vi "PicoScope2000aSettings.vi"(0 "error in":errorcluster, 1 "Channel A Settings":T2 {"Analogue Offset" format="%#_6p"; "Range" items=["20 mV", "50 mV", "100 mV", "200 mV", "500 mV", "1 V", "2 V", "5 V", "10 V", "20 V"]; "Coupling" items=["AC", "DC"]}, 3 "Channel B Settings":T2 {"Range" items=["20 mV", "50 mV", "100 mV", "200 mV", "500 mV", "1 V", "2 V", "5 V", "10 V", "20 V"]; "Coupling" items=["AC", "DC"]}, 5 "handle in":i16, 7 "Channel C Settings":T2 {"Analogue Offset" format="%#_6p"; "Range" items=["20 mV", "50 mV", "100 mV", "200 mV", "500 mV", "1 V", "2 V", "5 V", "10 V", "20 V"]; "Coupling" items=["AC", "DC"]}, 9 "Channel D Settings":T2 {"Analogue Offset" format="%#_6p"; "Range" items=["20 mV", "50 mV", "100 mV", "200 mV", "500 mV", "1 V", "2 V", "5 V", "10 V", "20 V"]; "Coupling" items=["AC", "DC"]}, 11 "Trigger Settings":T4 {"Trigger Direction" items=["Rising", "Falling"]}, 12 "Port 0 Settings":T3 {"Logic Level" items=["1.5V TTL", "2.5V CMOS"]}, 13 "Device Info":T1, 14 "Port 1 Settings":T3 {"Logic Level" items=["1.5V TTL", "2.5V CMOS"]}, 15 "Max_adc":i16) -> (4 "error out":errorcluster, 6 "handle out":i16, 8 "Enabled Array":i16[](array[numeric]))   [LabVIEW 2009]
doc: "This VI is used to set up the oscilloscope. The inputs are clusters for setting channel and simple trigger settings. Advanced triggers can be set up using PicoScope3000aAdvancedTriggerSettings.vi"
uses:
  ps2000a.dll
  PicoScope2000aAnalogChannelSettings.ctl
  PicoScope2000aDigitalChannelSettings.ctl
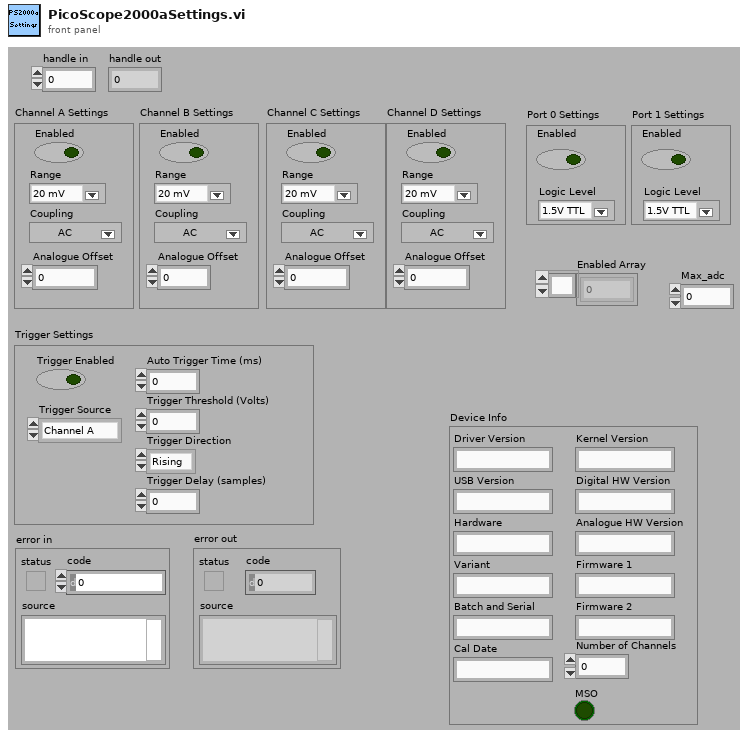
[diagram p1: front panel]
types:
  T1 = cluster{"Driver Version":string, "USB Version":string, "Hardware":string, "Variant":string, "Batch and Serial":string, "Cal Date":string, "Kernel Version":string, "Digital HW Version":string, "Analogue HW Version":string, "Firmware 1":string, "Firmware 2":string, "MSO":bool, "Number of Channels":i16}
  T2 = typedef "PicoScope2000aAnalogChannelSettings.ctl" = cluster{"Enabled":bool, "Coupling":i16, "Range":u16, "Analogue Offset":sgl}
  T3 = typedef "PicoScope2000aDigitalChannelSettings.ctl" = cluster{"Enabled":bool, "Logic Level":i16}
  T4 = cluster{"Trigger Enabled":bool, "Trigger Source":enum16{"Channel A", "Channel B", "Channel C", "Channel D", "Ext."}, "Trigger Threshold (Volts)":dbl, "Trigger Direction":u16, "Trigger Delay (samples)":u32, "Auto Trigger Time (ms)":i16}
  T5 = enum16{"Channel A", "Channel B", "Channel C", "Channel D", "Ext."}
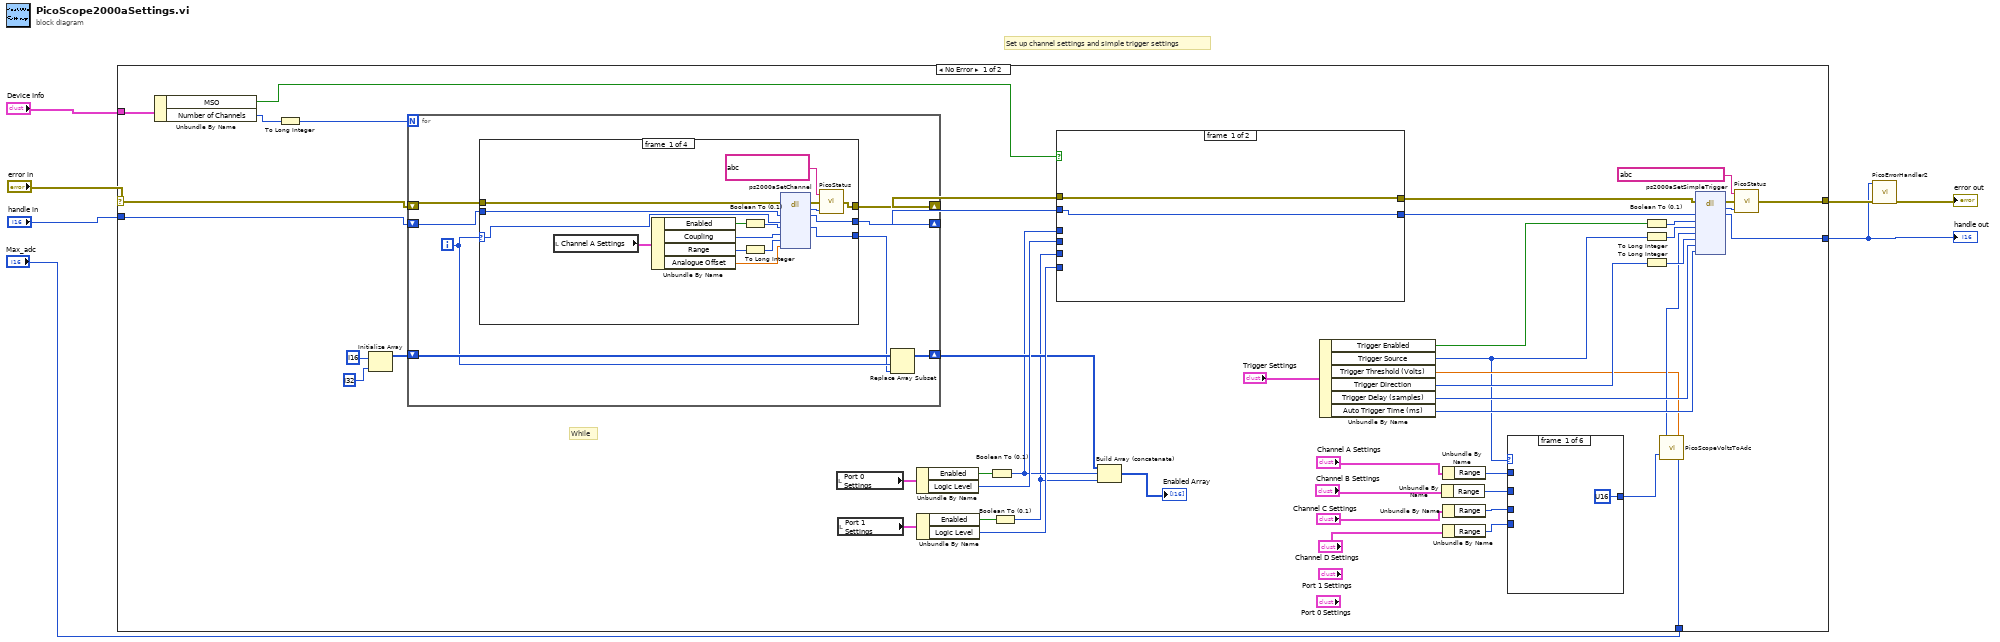
[diagram p0: block diagram]
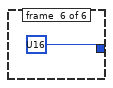
[diagram p6: hidden frame]
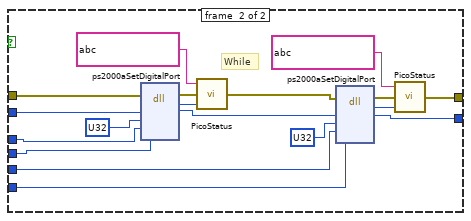
[diagram p7: hidden frame]
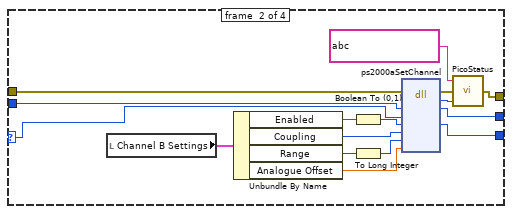
[diagram p8: hidden frame]
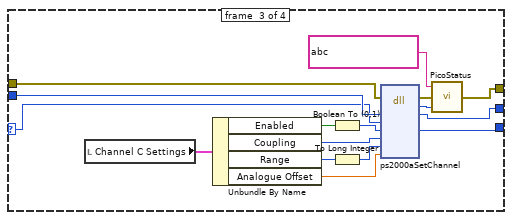
[diagram p9: hidden frame]
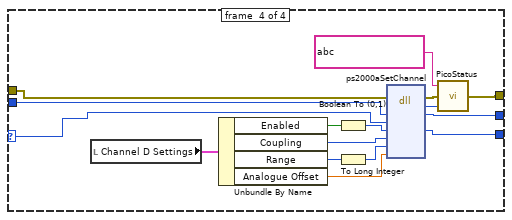
[diagram p10: hidden frame]
diagram:
  # "Set up channel settings and simple trigger settings"
  n1 = case shown="No Error" "error in" {
    selector: "error in" -> [w33 w155]
    tunnel: "handle in" -> [w32 w156]
    tunnel: [w9 w156] -> w2
    tunnel: "Max_adc" -> [w23 _]
    tunnel: "Device Info" -> [w25 _]
    tunnel: [w8 w155] -> w3
    frame #0 {
      # "While"
      n2 = Unbundle By Name(w25) -> ("MSO"=w24:bool, "Number of Channels"=w22:i16)
      n3 = To Long Integer(number=w22) -> (32bit integer=w11:i32)
      n4 = Initialize Array(i16 ? ("element"), i32 ? ("dimension size")) -> (w29:i16[])
      n5 = for {
        N: w11 -> [_]
        shift-right: [w90] -> w35
        shift-left: w33 -> [w89]
        shift-right: [w88] -> w34
        shift-left: w32 -> [w87]
        shift-right: [w83] -> w28
        shift-left: w29 -> [w86]
        i -> [w85]
        n6 = case shown="1" w85 {
          selector: w85 -> [w92 w108 w124 w140]
          tunnel: [w103 w119 w128 w144] -> w90
          tunnel: w89 -> [w102 w118 w126 w142]
          tunnel: w87 -> [w101 w117 w125 w141]
          tunnel: [w100 w116 w127 w143] -> w88
          tunnel: [w91 w107 w123 w139] -> w84
          frame #0 {
            n7 = local read "Channel A Settings"() -> (w93:T2)
            n8 = Unbundle By Name(w93) -> ("Enabled"=w96:bool, "Coupling"=w99:i16, "Range"=w94:u16, "Analogue Offset"=w98:sgl)
            n9 = Boolean To (0,1)(Boolean=w96) -> (0, 1=w97:i16)
            n10 = To Long Integer(number=w94) -> (32bit integer=w95:i32)
            n11 = dll-call lib="ps2000a.dll" fn="ps2000aSetChannel" ("ps2000a.dll:_ps3000_open_unit@0")(error in=w102, "handle"=w101, "channel"=w92, "enabled"=w97, "dc"=w99, "range"=w95, "analogueOffset"=w98) -> (error out=w105:errorcluster, "PICO_STATUS"=w104:u32, "handle"=w100:i16, "enabled"=w91:i16)  [unwired: 6 in, 1 out]
            n12 = call "PicoStatus.vi"("PICO STATUS"=w104, "error in"=w105, "source"=string ?) -> ("error out"=w103:errorcluster)
          }
          frame #1 {
            n13 = local read "Channel B Settings"() -> (w109:T2)
            n14 = Unbundle By Name(w109) -> ("Enabled"=w112:bool, "Coupling"=w115:i16, "Range"=w110:u16, "Analogue Offset"=w114:sgl)
            n15 = Boolean To (0,1)(Boolean=w112) -> (0, 1=w113:i16)
            n16 = To Long Integer(number=w110) -> (32bit integer=w111:i32)
            n17 = dll-call lib="ps2000a.dll" fn="ps2000aSetChannel" ("ps2000a.dll:_ps3000_open_unit@0")(error in=w118, "handle"=w117, "channel"=w108, "enabled"=w113, "dc"=w115, "range"=w111, "analogueOffset"=w114) -> (error out=w121:errorcluster, "PICO_STATUS"=w120:u32, "handle"=w116:i16, "enabled"=w107:i16)  [unwired: 6 in, 1 out]
            n18 = call "PicoStatus.vi"("PICO STATUS"=w120, "error in"=w121, "source"=string ?) -> ("error out"=w119:errorcluster)
          }
          frame #2 {
            n19 = local read "Channel C Settings"() -> (w138:T2)
            n20 = Unbundle By Name(w138) -> ("Enabled"=w135:bool, "Coupling"=w132:i16, "Range"=w137:u16, "Analogue Offset"=w133:sgl)
            n21 = Boolean To (0,1)(Boolean=w135) -> (0, 1=w134:i16)
            n22 = To Long Integer(number=w137) -> (32bit integer=w136:i32)
            n23 = dll-call lib="ps2000a.dll" fn="ps2000aSetChannel" ("ps2000a.dll:_ps3000_open_unit@0")(error in=w126, "handle"=w125, "channel"=w124, "enabled"=w134, "dc"=w132, "range"=w136, "analogueOffset"=w133) -> (error out=w130:errorcluster, "PICO_STATUS"=w131:u32, "handle"=w127:i16, "enabled"=w123:i16)  [unwired: 6 in, 1 out]
            n24 = call "PicoStatus.vi"("PICO STATUS"=w131, "error in"=w130, "source"=string ?) -> ("error out"=w128:errorcluster)
          }
          frame #3 {
            n25 = local read "Channel D Settings"() -> (w154:T2)
            n26 = Unbundle By Name(w154) -> ("Enabled"=w151:bool, "Coupling"=w148:i16, "Range"=w153:u16, "Analogue Offset"=w149:sgl)
            n27 = Boolean To (0,1)(Boolean=w151) -> (0, 1=w150:i16)
            n28 = To Long Integer(number=w153) -> (32bit integer=w152:i32)
            n29 = dll-call lib="ps2000a.dll" fn="ps2000aSetChannel" ("ps2000a.dll:_ps3000_open_unit@0")(error in=w142, "handle"=w141, "channel"=w140, "enabled"=w150, "dc"=w148, "range"=w152, "analogueOffset"=w149) -> (error out=w146:errorcluster, "PICO_STATUS"=w147:u32, "handle"=w143:i16, "enabled"=w139:i16)  [unwired: 6 in, 1 out]
            n30 = call "PicoStatus.vi"("PICO STATUS"=w147, "error in"=w146, "source"=string ?) -> ("error out"=w144:errorcluster)
          }
        }
        n31 = Replace Array Subset(array=w86, new element=w84, index=w85) -> (w83:i16[])
      }
      n32 = local read "Port 0 Settings"() -> (w42:T3)
      n33 = local read "Port 1 Settings"() -> (w40:T3)
      n34 = Unbundle By Name(w42) -> ("Enabled"=w43:bool, "Logic Level"=w39:i16)
      n35 = Unbundle By Name(w40) -> ("Enabled"=w41:bool, "Logic Level"=w38:i16)
      n36 = Boolean To (0,1)(Boolean=w43) -> (0, 1=w27:i16)
      n37 = Boolean To (0,1)(Boolean=w41) -> (0, 1=w26:i16)
      n38 = case shown="True" w24 {
        tunnel: w27 -> [_ w74]
        tunnel: w39 -> [_ w73]
        tunnel: w26 -> [_ w72]
        tunnel: w38 -> [_ w71]
        tunnel: [w64 w68] -> w37
        tunnel: [w63 w67] -> w36
        tunnel: w35 -> [w64 w66]
        tunnel: w34 -> [w63 w65]
        frame #0 {
        }
        frame #1 {
          # "While"
          n39 = dll-call lib="PS2000a.dll" fn="ps2000aSetDigitalPort"(error in=w66, "handle"=w65, "port"=u32 ? ("channel"), "enabled"=w74, "logicLevel"=w73) -> (error out=w82:errorcluster, "PICO_STATUS"=w80:u32, "handle"=w70:i16)  [unwired: 5 in, 1 out]
          n40 = call "PicoStatus.vi"("PICO STATUS"=w80, "error in"=w82, "source"=string ?) -> ("error out"=w69:errorcluster)
          n41 = dll-call lib="PS2000a.dll" fn="ps2000aSetDigitalPort"(error in=w69, "handle"=w70, "port"=u32 ? ("channel"), "enabled"=w72, "logicLevel"=w71) -> (error out=w78:errorcluster, "PICO_STATUS"=w76:u32, "handle"=w67:i16)  [unwired: 5 in, 1 out]
          n42 = call "PicoStatus.vi"("PICO STATUS"=w76, "error in"=w78, "source"=string ?) -> ("error out"=w68:errorcluster)
        }
      }
      n43 = Build Array (concatenate)(w28, w27, w26) -> (→"Enabled Array":i16[])
      n44 = Unbundle By Name("Trigger Settings") -> ("Trigger Enabled"=w50:bool, "Trigger Source"=w20:T5, "Trigger Threshold (Volts)"=w44:dbl, "Trigger Direction"=w53:u16, "Trigger Delay (samples)"=w52:u32, "Auto Trigger Time (ms)"=w51:i16)
      n45 = Unbundle By Name("Channel B Settings") -> ("Range"=w18:u16)
      n46 = Unbundle By Name("Channel A Settings") -> ("Range"=w19:u16)
      n47 = Unbundle By Name("Channel C Settings") -> ("Range"=w17:u16)
      n48 = Unbundle By Name("Channel D Settings") -> ("Range"=w16:u16)
      n49 = case shown="\"Channel A\"" w20 {
        tunnel: [u16 ? ("Range") w58 w59 w60 w61 u16 ? ("Range")] -> w21
        tunnel: w19 -> [_ w58 _ _ _ _]
        tunnel: w18 -> [_ _ w59 _ _ _]
        tunnel: w17 -> [_ _ _ w60 _ _]
        tunnel: w16 -> [_ _ _ _ w61 _]
        frame #0 {
        }
        frame #1 {
        }
        frame #2 {
        }
        frame #3 {
        }
        frame #4 {
        }
        frame #5 {
        }
      }
      n50 = Boolean To (0,1)(Boolean=w50) -> (0, 1=w49:i16)
      n51 = To Long Integer(number=w20) -> (32bit integer=w56:i32)
      n52 = To Long Integer(number=w53) -> (32bit integer=w55:i32)
      n53 = call "PicoScopeVoltsToAdc.vi"("Max_adc"=w23, "Volts"=w44, "Range Index"=w21) -> ("ADC count"=w45:i16)
      n54 = dll-call lib="ps2000a.dll" fn="ps2000aSetSimpleTrigger" ("ps2000a.dll:_ps3000_open_unit@0")(error in=w37, "handle"=w36, "enabled"=w49, "source"=w56, "threshold"=w45, "direction"=w55, "delay"=w52, "autoTrigger_ms"=w51) -> (error out=w47:errorcluster, "PICO_STATUS"=w48:u32, "handle"=w9:i16)  [unwired: 8 in, 1 out]
      n55 = call "PicoStatus.vi"("PICO STATUS"=w48, "error in"=w47, "source"=string ?) -> ("error out"=w8:errorcluster)
    }
    frame #1 {
    }
  }
  "handle out" <- w2
  n56 = call "PicoErrorHandler2.vi"("error in (no error)"=w3, "handle In"=w2) -> ("error out"=→"error out":errorcluster)  [unwired: 9 in]
